vi "FuncVI-QueueCreate.vi"(5 "InstanceRef":T2, 9 "arg list":T1[](array[typedef]) {"num" format="%.2f"}) -> (0 "error out":bool, 3 "result":T1 {"num" format="%.2f"})   [LabVIEW 2021]
doc: "::: CalcExpress Toolkit :::\nCopyright (c) 2000-2026 Konstantin Shifershteyn. All rights reserved."
uses:
  cetypes.llb/CalcExpress Function Argument Info.ctl
  cetypes.llb/CalcExpress Instance RefNum.ctl
panel:
  in  "max arg num":i32=2
  in  "min arg num":i32=1
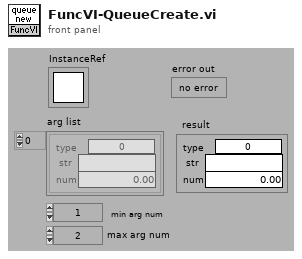
[diagram p1: front panel]
types:
  T1 = typedef "CalcExpress Function Argument Info.ctl" = cluster{"type":u32, "str":string, "num":dbl}
  T2 = typedef "CalcExpress Instance RefNum.ctl" = refnum<k1>
  T3 = cluster{"index":i32, "data type":enum32{"String", "DBL Number", "identifier", "1D Array of DBL", "2D Array of DBL", "CDB Number", "1D Array of CDB", "2D Array of CDB", "1D Array of String", "2D Array of String", "Unknown data type"}, "default num":dbl, "default str":string}[]
  T4 = enum32{"String", "DBL Number", "identifier", "1D Array of DBL", "2D Array of DBL", "CDB Number", "1D Array of CDB", "2D Array of CDB", "1D Array of String", "2D Array of String", "Unknown data type"}
  T5 = cluster{"data type":enum32{"String", "DBL Number", "identifier", "1D Array of DBL", "2D Array of DBL", "CDB Number", "1D Array of CDB", "2D Array of CDB", "1D Array of String", "2D Array of String", "Unknown data type"}, string, dbl}
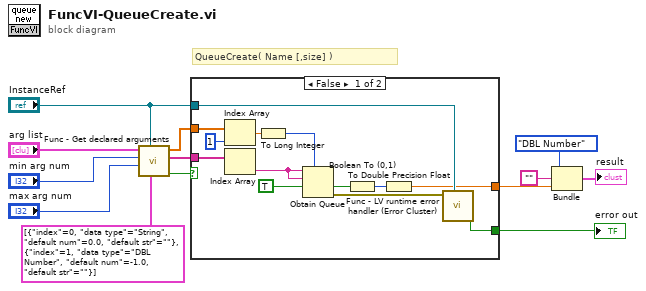
[diagram p0: block diagram]
diagram:
  # "QueueCreate( Name [,size] )"
  n1 = call "Func - Get declared arguments.vi"("arg descriptors"=T3 [{"index"=0, "data type"=enum."String", "default num"=0.0, "default str"=""}, {"index"=1, "data type"=enum."DBL Number", "default num"=-1.0, "default str"=""}], "InstanceRef"="InstanceRef", "max arg num"="max arg num", "min arg num"="min arg num", "arg list"="arg list") -> ("error out"=w5:bool, "str list"=w12:string[], "num list"=w6:dbl[])  [unwired: 3 in, 1 out]
  n2 = case shown="False" w5 {
    selector: w5 -> [_ w27]
    tunnel: w12 -> [w26 _]
    tunnel: "InstanceRef" -> [w20 _]
    tunnel: w6 -> [w23 _]
    tunnel: [w19 w27] -> w4
    tunnel: [w14 _] -> w1
    frame False {
      n3 = Index Array(array=w23, index=1) -> (element=w22:dbl)
      n4 = Index Array(array=w26) -> (element=w17:string)  [unwired: 1 in]
      n5 = To Long Integer(number=w22) -> (32bit integer=w18:i32)
      n6 = Obtain Queue(max queue size (-1, unlimited)=w18, name (unnamed)=w17, element data type=w17, create if not found? (T)=TRUE ("return exisiting (F)")) -> (created new?=w16:bool, error out=w21:errorcluster)  [unwired: 1 in, 1 out]
      n7 = Boolean To (0,1)(Boolean=w16) -> (0, 1=w15:i16)
      n8 = To Double Precision Float(number=w15) -> (double precision float=w14:dbl)
      n9 = call "Func - LV runtime error handler (Error Cluster).vi"("InstanceRef"=w20, "LabVIEW error"=w21) -> ("error out"=w19:bool)  [unwired: 4 in, 3 out]
    }
    frame True {
    }
  }
  "error out" <- w4
  n10 = Bundle("data type"=T4."DBL Number", "", w1) -> (→"result":T5)  [unwired: 1 in]
